vi "Destroy.vi"(0 "ClassWriterGOOP300.lvclass":refnum<class "ClassWriterGOOP400.lvclass">, 5 "error in (no error)":errorcluster) -> (19 "error out":errorcluster)   [LabVIEW 2020, in "ClassWriterGOOP400.lvclass"]
doc: "Destroys a ClassWriterNative object created with a ClassWriterNative constructor VI.\n\n[GOOP 2.0.16]"
uses:
  ClassWriterGOOP400.lvclass
  Provider_EndevoGOOP300/ClassWriterGOOP300_class/ClassWriterGOOP300.lvclass
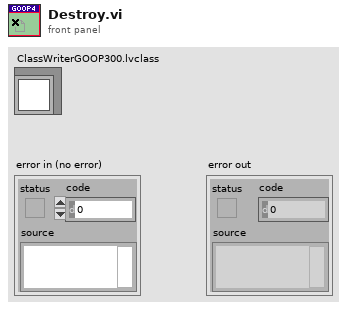
[diagram p1: front panel]
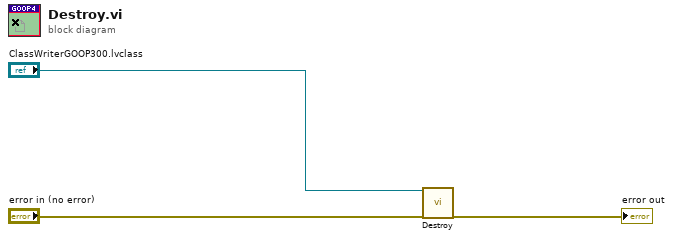
[diagram p0: block diagram]
diagram:
  n1 = call-parent "Destroy.vi"("ClassWriterGOOP300.lvclass"="ClassWriterGOOP300.lvclass", "error in (no error)"="error in (no error)") -> ("error out"=→"error out":errorcluster)  [unwired: 17 in]
